vi "Send Data.vi"(7 "Finished Late":bool, 8 "error in (no error)":errorcluster, 11 "ValveControlModule in":refnum<class "DigitalControlModule.lvclass">) -> (0 "error out":errorcluster, 3 "ValveControlModule out":refnum<class "DigitalControlModule.lvclass">)   [LabVIEW 2020, in "VolatusControl.lvlib" / "DigitalControlModule.lvclass"]
uses:
  DigitalControlModule.lvclass
  DigitalControlModule.lvclass/DigitalControlModule.ctl
  VolatusData/Data Buffer DBL/Data Buffer DBL.lvclass
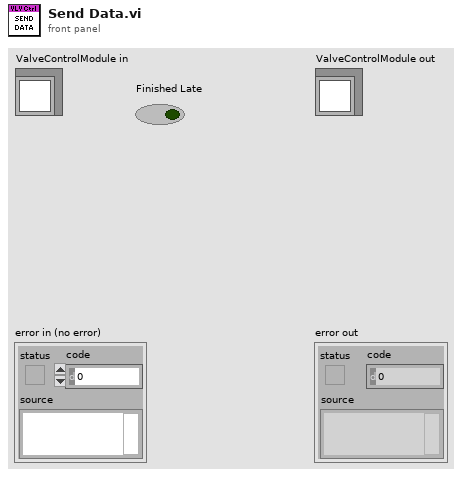
[diagram p1: front panel]
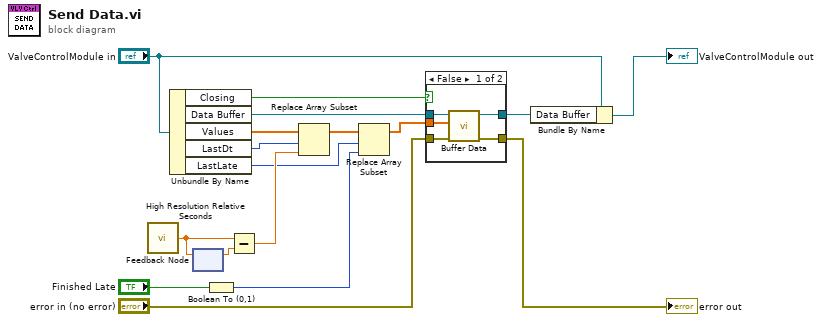
[diagram p0: block diagram]
diagram:
  n1 = call <vilib>:"High Resolution Relative Seconds.vi"() -> ("relative seconds"=w14:dbl)
  n2 = Unbundle By Name("ValveControlModule in") -> ("Closing"=w1:bool, "Data Buffer"=w7:refnum<class "Data Buffer DBL.lvclass">, "Values"=w16:dbl[], "LastDt"=w11:i32, "LastLate"=w9:i32)
  n3 = feedback #1() -> (w15:dbl)  [unwired: 1 in]
  n4 = feedback-in #1(w14) -> ()
  n5 = Boolean To (0,1)(Boolean="Finished Late") -> (0, 1=w8:i16)
  n6 = Subtract(x=w14, y=w15) -> (x-y=w10:dbl)
  n7 = Replace Array Subset(array=w16, new element=w10, index=w11) -> (w12:dbl[])
  n8 = Replace Array Subset(array=w12, new element=w8, index=w9) -> (w6:dbl[])
  n9 = case shown="False" w1 {
    tunnel: w7 -> [w22 w24]
    tunnel: w6 -> [w21 _]
    tunnel: "error in (no error)" -> [w20 w23]
    tunnel: [w19 w23] -> w4
    tunnel: [w18 w24] -> w2
    frame False {
      n10 = call "Buffer Data.vi"("error in (no error)"=w20, "Data"=w21, "Data Buffer in"=w22) -> ("error out"=w19:errorcluster, "Data Buffer out"=w18:refnum<class "Data Buffer DBL.lvclass">)  [unwired: 7 in]
    }
    frame True {
    }
  }
  "error out" <- w4
  n11 = Bundle By Name(cluster="ValveControlModule in", "Data Buffer"=w2) -> (→"ValveControlModule out":refnum<class "DigitalControlModule.lvclass">)
